vi "query Axis Parameter List.vi"(8 "error in (no error)":errorcluster, 11 "3D Controller in":refnum<class "3D Controller.lvclass">) -> (0 "error out":errorcluster, 1 "Valid":bool, 2 "Axis Parameter List":T1, 3 "3D Controller out":refnum<class "3D Controller.lvclass">)   [LabVIEW 2023, in "FCC 3D Controller for BS.lvlib" / "3D Controller.lvclass"]
uses:
  3D Controller.lvclass
  Type Definition/TYPE Axis Parameter List.ctl
  3D Controller.lvclass/3D Controller.ctl
  FCC 3D Controller for BS.lvlib
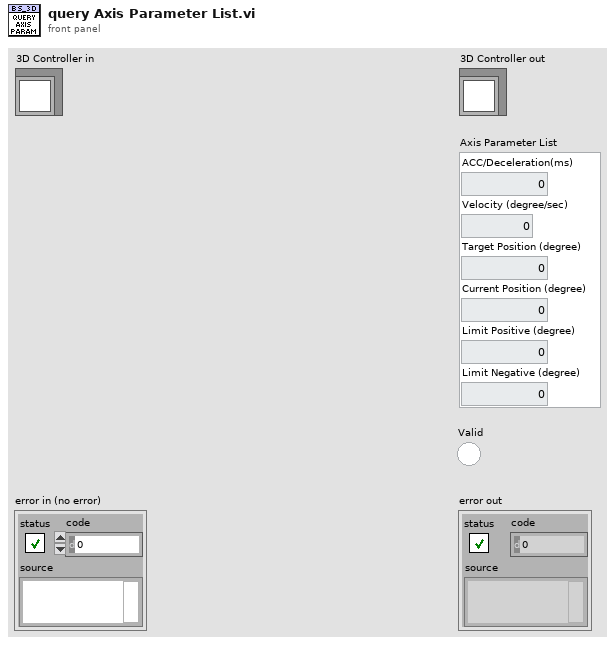
[diagram p1: front panel]
types:
  T1 = typedef "FCC 3D Controller for BS.lvlib/TYPE Axis Parameter List.ctl" = cluster{"ACC/Deceleration(ms)":dbl, "Velocity (degree/sec)":dbl, "Target Position (degree)":dbl, "Current Position (degree)":dbl, "Limit Positive (degree)":dbl, "Limit Negative (degree)":dbl}
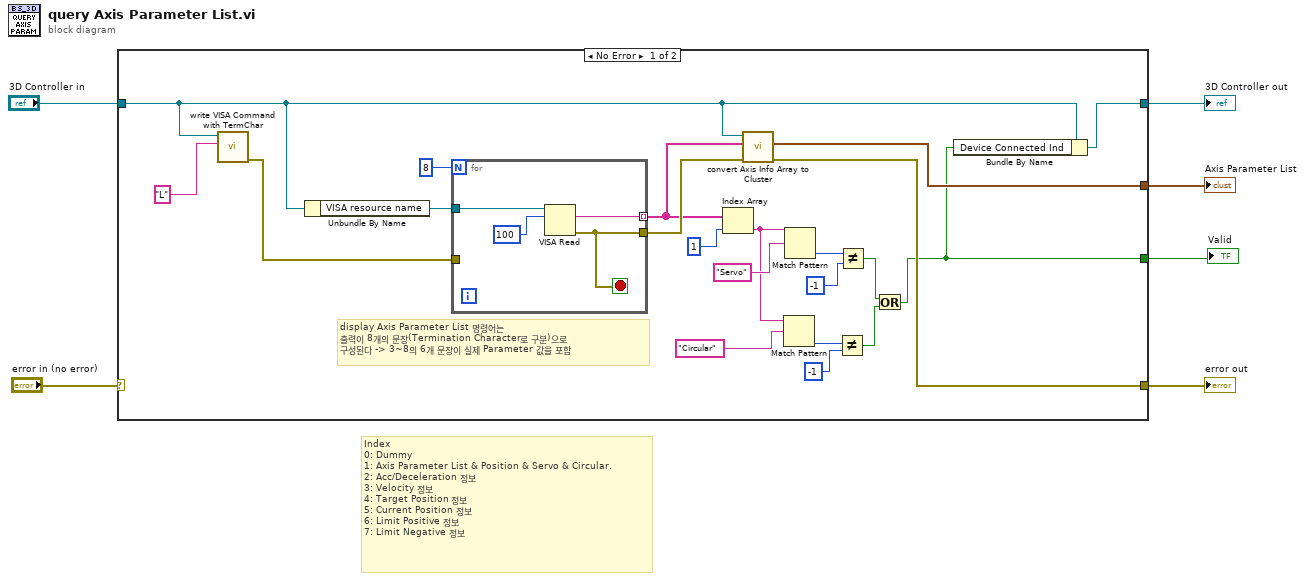
[diagram p0: block diagram]
diagram:
  # "Index\n0: Dummy\n1: Axis Parameter List & Position & Servo & Circular.\n2: Acc/Deceleration 정보\n3: Velocity 정보\n4: Target Position 정보\n5: Current Position 정보\n6: Limit Positive 정보\n7: Limit Negative 정보"
  n1 = case shown="No Error" "error in (no error)" {
    selector: "error in (no error)" -> [_ w33]
    tunnel: "3D Controller in" -> [w15 w32]
    tunnel: [w22 w33] -> w4
    tunnel: [w14 w32] -> w3
    tunnel: [w23 _] -> w2
    tunnel: [w7 _] -> w1
    frame No Error {
      # "display Axis Parameter List 명령어는\n출력이 8개의 문장(Termination Character로 구분)으로\n구성된다 -> 3~8의 6개 문장이 실제 Parameter 값을 포함"
      n2 = call "write VISA Command with TermChar.vi"("Command String"="L", "3D Controller in"=w15) -> ("error out"=w16:errorcluster)  [unwired: 8 in, 1 out]
      n3 = Unbundle By Name(w15) -> ("VISA resource name"=w26:refnum<visa-resource-name>)
      n4 = for {
        N: 8 -> [_]
        tunnel: w26 -> [w31]
        tunnel: [w29] -> w21 mode=indexing
        tunnel: [w28] -> w24
        tunnel: w16 -> [_]
        stop <- w28 stop-if-true
        n5 = VISA Read(VISA resource name=w31, byte count=u32 100) -> (read buffer=w29:string, error out=w28:errorcluster)  [unwired: 1 in, 2 out]
      }
      n6 = Index Array(array=w21, index=1) -> (element=w13:string)
      n7 = call "convert Axis Info Array to Cluster.vi"("error in (no error)"=w24, "Axis Info Array"=w21, "3D Controller in"=w15) -> ("error out"=w22:errorcluster, "Axis Parameter List"=w23:T1)  [unwired: 6 in, 1 out]
      n8 = Match Pattern(string=w13, regular expression="Circular") -> (offset past match=w11:i32)  [unwired: 1 in, 3 out]
      n9 = Match Pattern(string=w13, regular expression="Servo") -> (offset past match=w18:i32)  [unwired: 1 in, 3 out]
      n10 = Not Equal?(x=w11, y=-1) -> (x != y?=w8:bool)
      n11 = Not Equal?(x=w18, y=-1) -> (x != y?=w9:bool)
      n12 = Or(x=w9, y=w8) -> (x .or. y?=w7:bool)
      n13 = Bundle By Name(cluster=w15, "Device Connected Ind"=w7) -> (w14:refnum<class "3D Controller.lvclass">)
    }
    frame Error {
    }
  }
  "error out" <- w4
  "3D Controller out" <- w3
  "Valid" <- w1
  "Axis Parameter List" <- w2
